vi "Migrate Measurements.vi"() -> ()   [LabVIEW 2021]
uses:
  _Measurement Migrator/Migrator/Queue Driver/controls/Queue Operations.ctl
  _Measurement Migrator/Migrator/Migration Logic/controls/Multiple Migration/Multiple Migration Data Holder.ctl
  <vilib>/Utility/sysdir.llb/System Directory Type.ctl
  <vilib>/Utility/miscctls.llb/LVRowAndColumnUnsignedTypeDef.ctl
  <vilib>/Utility/miscctls.llb/LVRowAndColumnTypeDef.ctl
  _Measurement Migrator/Migrator/Migrator Reusables/controls/Dictionary States.ctl
  <vilib>/Utility/cursorutil.llb/Set Cursor (Icon Pict).vi
  _Measurement Migrator/Migrator/Queue Driver/Queue Driver.lvlib
  _Measurement Migrator/Migrator/Migration Logic/Migrator.lvlib
  _Measurement Migrator/Migrator/Path Functions/Path Functions.lvlib
  _Measurement Migrator/Migrator/Multiple Migrator/Multiple Migrator.lvlib
  _Measurement Migrator/Migrator/Migrator Reusables/Migrator Reusables.lvlib
panel:
  out "error out":errorcluster
  in  "Tab Control":T1(tab)
  in  "Info":string
  in  "Select Measurement":path
  out "Warning":bool=TRUE caption="Warning:\nMeasurement should be an existing VI or folder path"
  in  "Populate measurements":bool
  in  "Select Project":path=path "C:/Users/aishwarya.lakshmi/Documents/Measurement Plug-ins/Measurement"
  in  "Select all":bool
  in  "Back to Home":bool
  in  "List Plug-ins":bool
  in  "Select Measurements":string(tree)
  out "Selection warning":string="Atleast one measurement should be selected"
  out "Plug-in info":string="* Rename the Plug-in if required"
  out "Plug-in warning":string="Warning:\n1. Measurement plug-in name must be unique \n2. Plugin name cannot contain any of the following characters:\n         \\ / : * ? \" < > |"
  in  "Start Migration":bool
  in  "Back to Select":bool
  in  "List of Selected Measurements":i32(listbox)
  in  "Measurement Count":i32(slide)=6 caption="Migrating 1 of 1 measurement(s)" scale=0.0..100.0
  in  "Progress":i32(slide)=9 caption="Saving the project files..." scale=0.0..15.0
  in  "Review":bool
  in  "Migration Status":i32(listbox)
  in  "Back to Status":bool
  in  "Select Plug-in":string(combo) caption="Select Measurement plug-in to review"
  in  "Start Next":bool
  out "Launch Type Spec":string
  out "Launch Logic":string
  out "Launch UI":string
  # "* Project in which the measurement plug-in will be created"
  # "* Select a measurement vi or a folder containing measurements"
  # ".lvproj"
  # "Select the measurements to migrate"
  # "Review the Measurement:\n1. Review the Measurement UI. Click here to launch.\n2. Review the Measurement Logic VI. Click here to launch.\n3. Review the Type Specialization VI. Click here to launch."
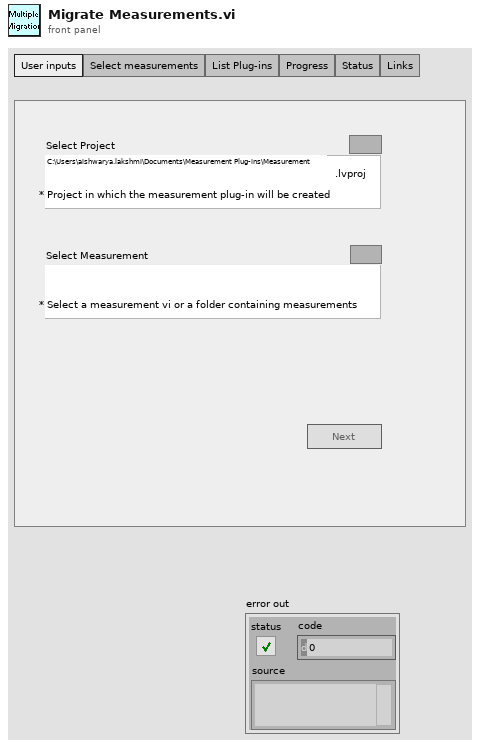
[diagram p1: front panel]
types:
  T1 = enum32{"User inputs", "Select measurements", "List Plug-ins", "Progress", "Status", "Links"}
  T2 = typedef "Queue Driver.lvlib/Queue Operations.ctl" = enum16{"Create Q", "Enqueue", "Enqueue N", "Dequeue", "Flush", "Release"}
  T3 = typedef "Migrator.lvlib/Multiple Migration Data Holder.ctl" = cluster{"Tree Reference":refnum<vi>, "LabVIEW Version":string, "Project path":path, "Create new project?":bool, "Measurement file/folder path":path, "Measurement folder selected?":bool, "Project warning":string, "Measurement warning":string, "Next clicked?":bool, "Measurement path changed?":bool, "Select all":bool, "Measurement folder Tags":string[], "Measurement file Tags":string[], "Selected cell Tag":string, "Measurement Plug-ins":string[][], "Measurement File Paths":path[], "Plugin Migration Value":i32, "Migration Count":i32, "Instrument containing subVIs":path[][], "Progress per measurement":i32, "Measurement Progress":i32, "Migration Status":string[][]}
  T4 = enum8{"Enabled", "Disabled", "Disabled and Grayed Out"}
  T5 = typedef "LVRowAndColumnUnsignedTypeDef.ctl" = cluster{"Row":u32, "Column":u32}
  T6 = typedef "LVRowAndColumnTypeDef.ctl" = cluster{"Row":i32, "Column":i32}
  T7 = typedef "Migrator Reusables.lvlib/Dictionary States.ctl" = enum16{"Set", "Get", "Delete", "Delete All"}
  T8 = typedef "System Directory Type.ctl" = i32
  T9 = typedef "LVPoint32TypeDef.ctl" = cluster{"Horizontal":i32, "Vertical":i32}
  T10 = typedef "Migrator.lvlib/Tree Items.ctl" = cluster{"Item name":string, "Indent":i32, "Tag":string}
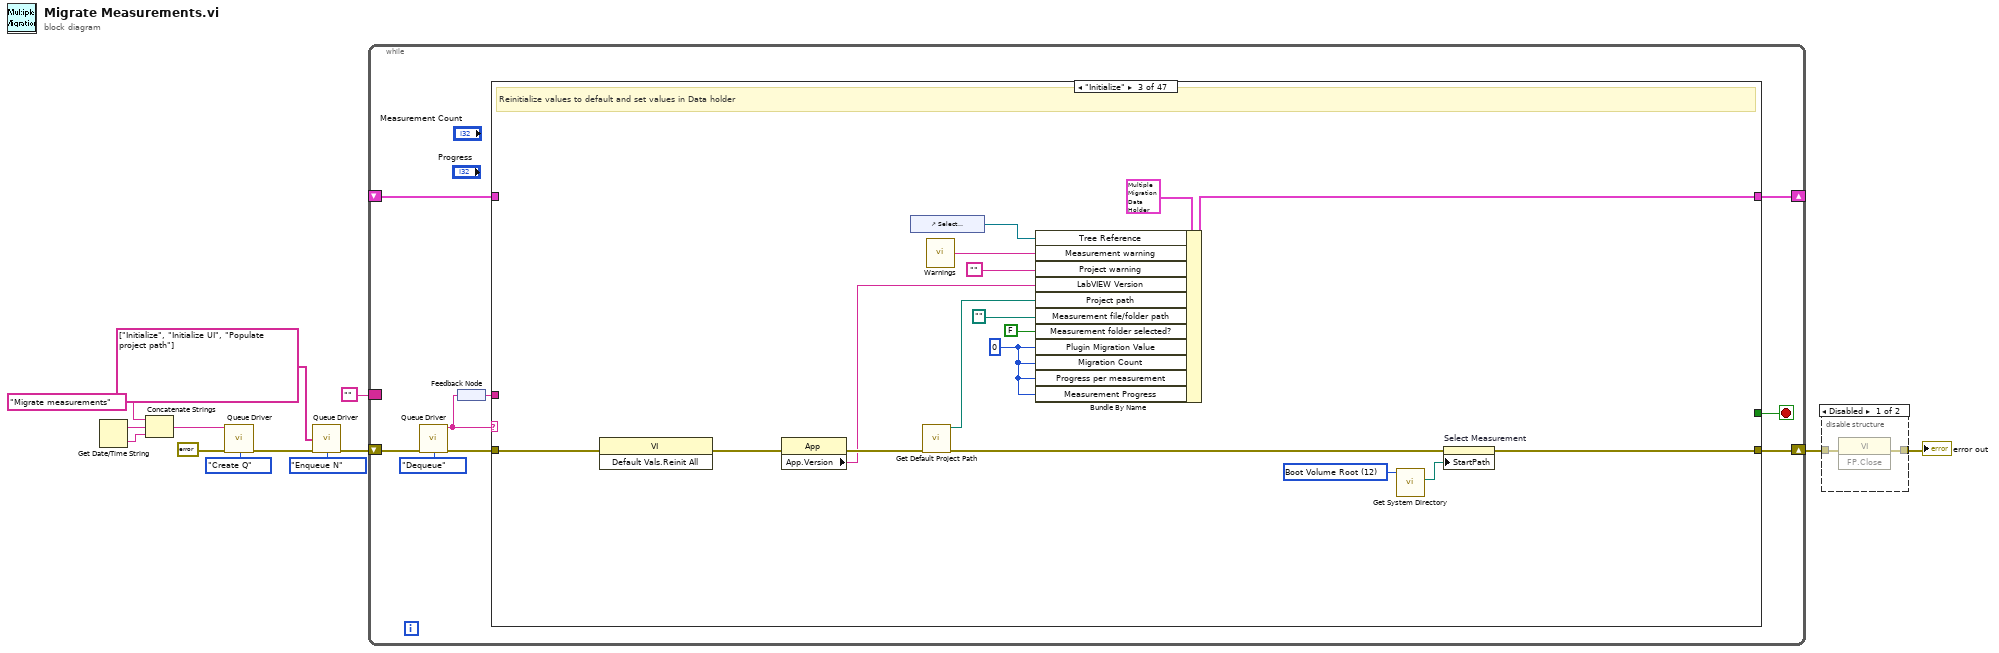
[diagram p0: block diagram]
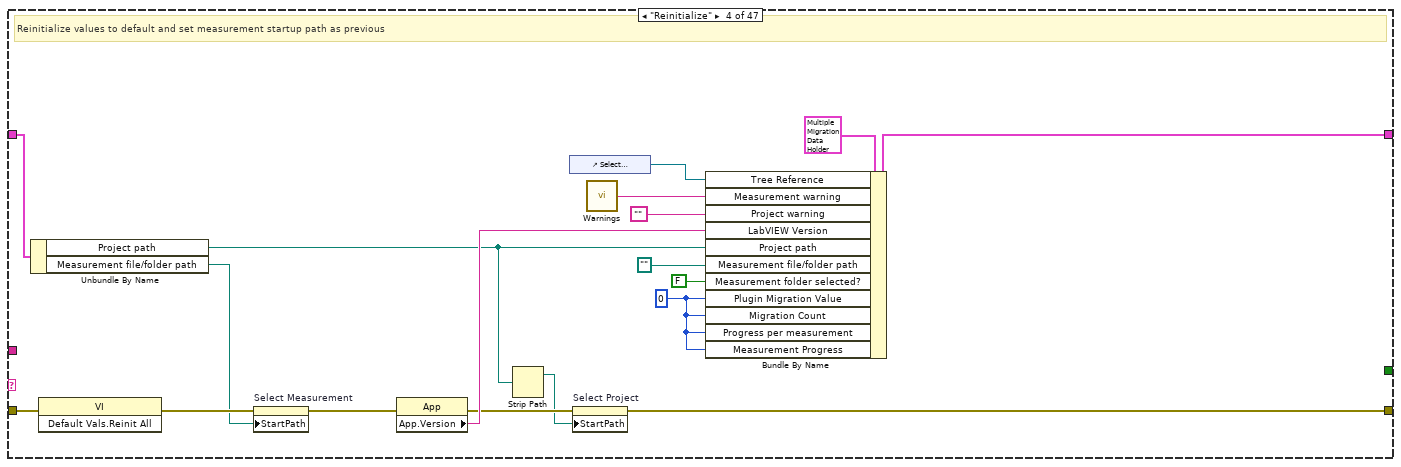
[diagram p5: hidden frame]
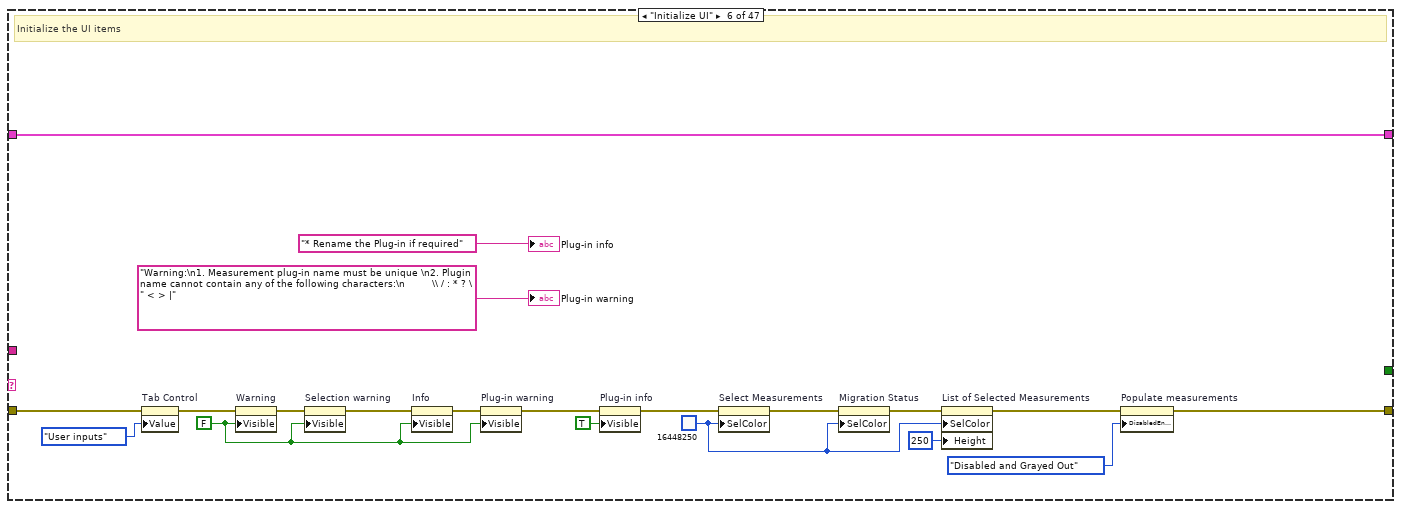
[diagram p7: hidden frame]
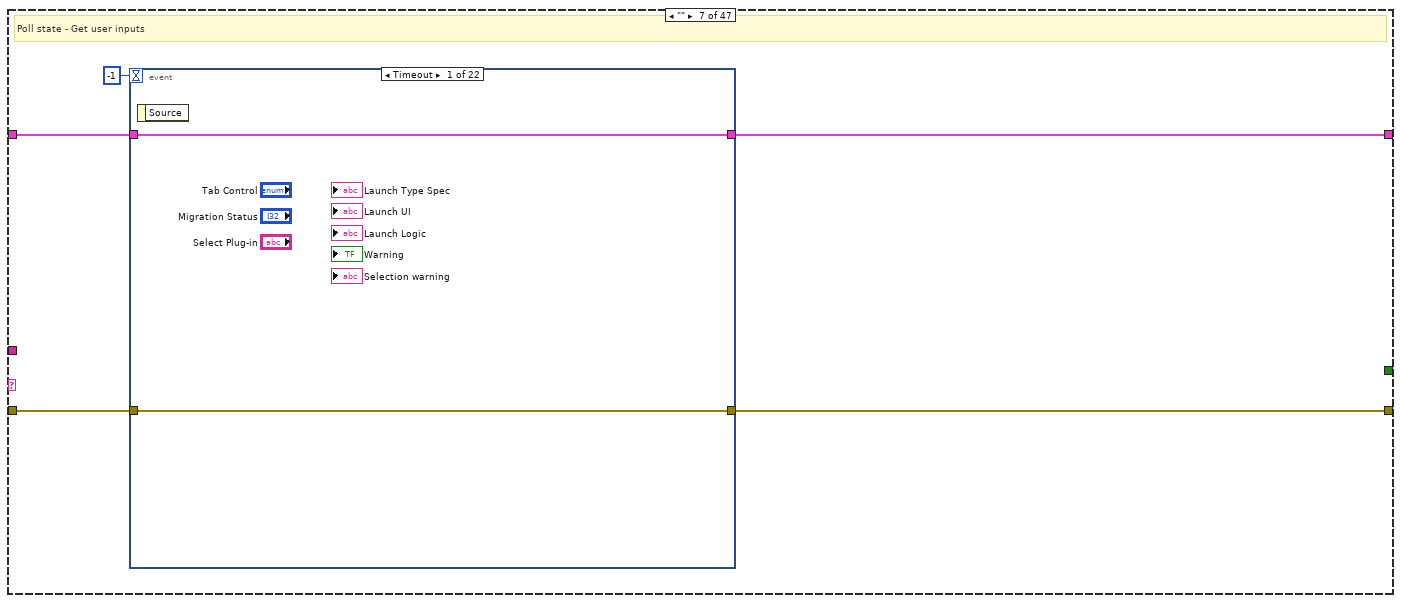
[diagram p8: hidden frame]
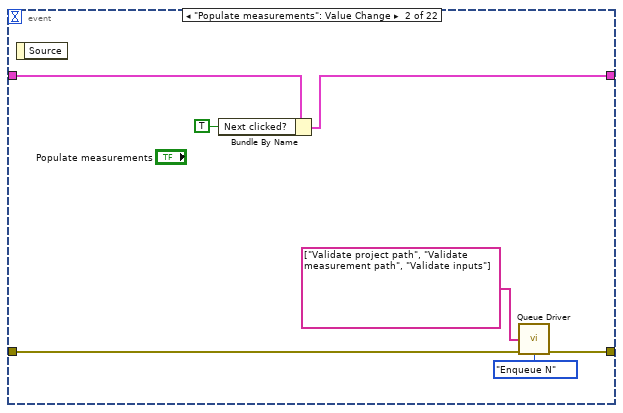
[diagram p9: hidden frame]
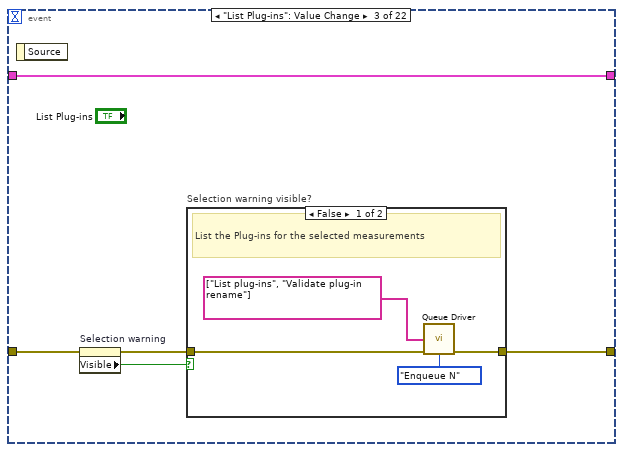
[diagram p10: hidden frame]
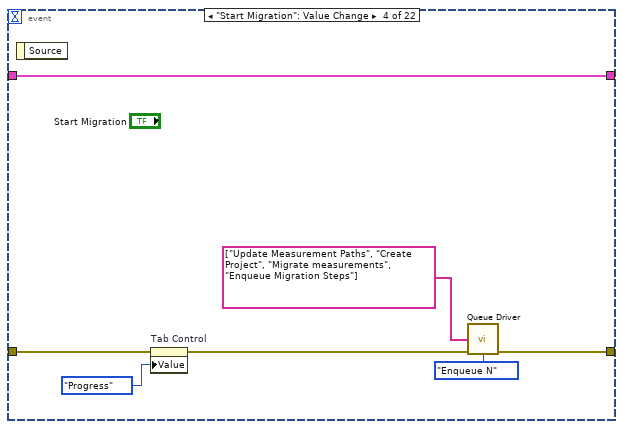
[diagram p12: hidden frame]
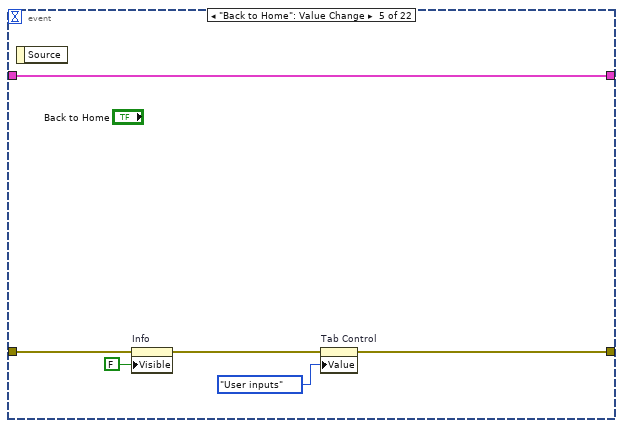
[diagram p13: hidden frame]
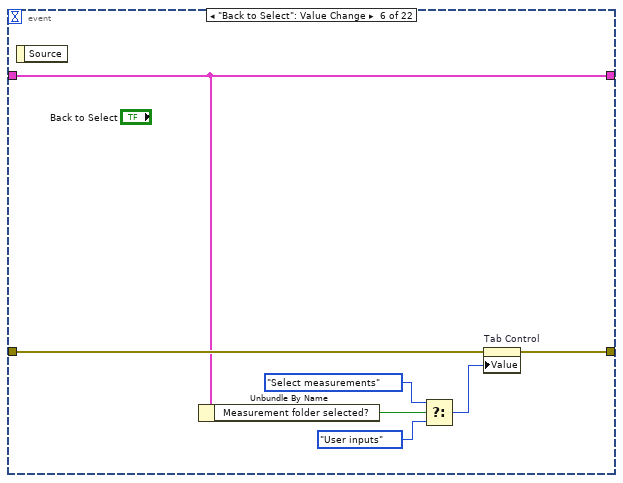
[diagram p14: hidden frame]
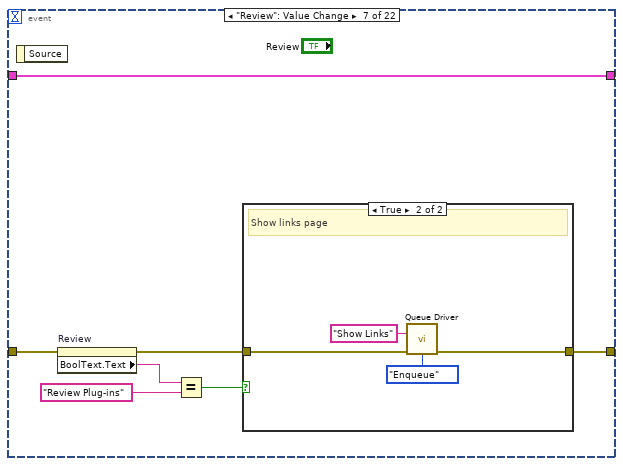
[diagram p15: hidden frame]
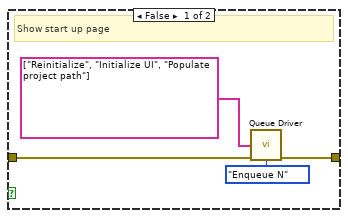
[diagram p16: hidden frame]
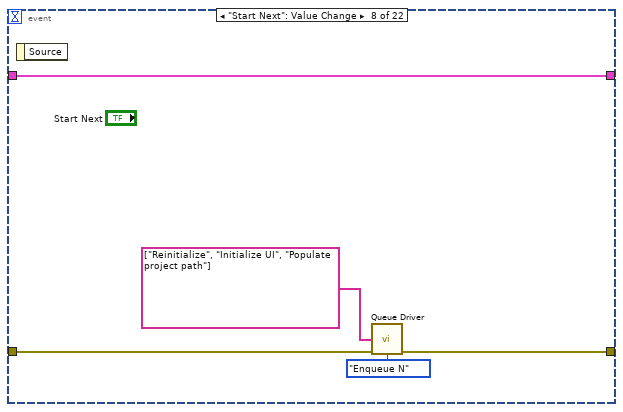
[diagram p17: hidden frame]
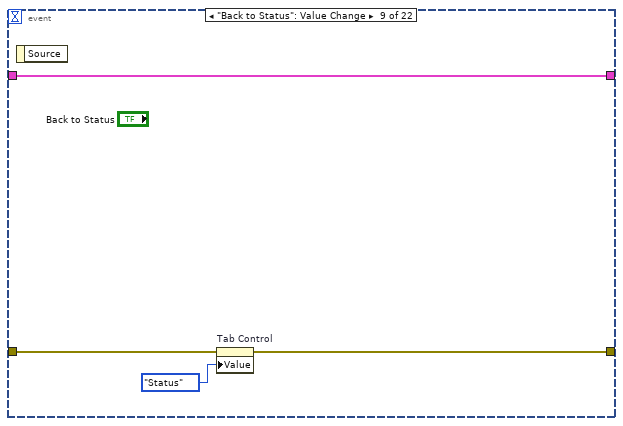
[diagram p18: hidden frame]
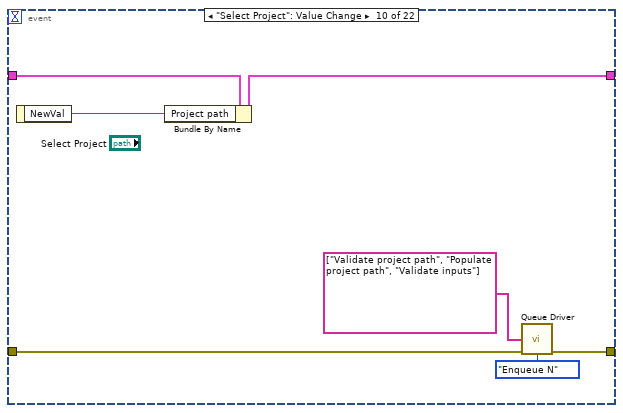
[diagram p19: hidden frame]
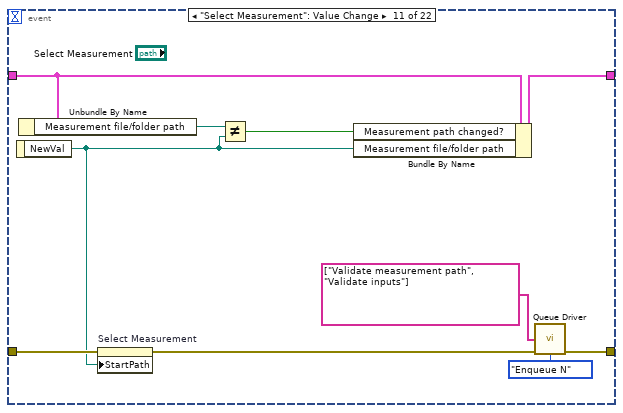
[diagram p20: hidden frame]
diagram:
  n1 = Get Date/Time String() -> (date string=w10:string, time string=w9:string)  [unwired: 3 in]
  n2 = Concatenate Strings("Migrate measurements" ("string"), w10, w9) -> (w4:string)
  n3 = call "Queue Driver.vi"("Name"=w4, "error in (no error)"=errorcluster {"status"=FALSE, "code"=0, "source"=""}, "Q Operations"=Queue_Operations."Create Q") -> ("error out"=w13:errorcluster)  [unwired: 11 in, 1 out]
  n4 = call "Queue Driver.vi"("States[]"=string[] ["Initialize", "Initialize UI", "Populate project path"], "error in (no error)"=w13, "Q Operations"=Queue_Operations."Enqueue N") -> ("error out"=w8:errorcluster)  [unwired: 11 in, 1 out]
  n5 = while {
    shift-right: [w21] -> w3
    shift-left: w8 -> [w22]
    shift-right: [w18] -> _
    shift-left: _ -> [w17]
    border: "" -> [_]
    stop <- w16 stop-if-true
    n6 = call "Queue Driver.vi"("error in (no error)"=w22, "Q Operations"=Queue_Operations."Dequeue") -> ("Dequeued State"=w15:string, "error out"=w20:errorcluster)  [unwired: 12 in]
    n7 = feedback #1() -> (w14:string)
    n8 = feedback-in #1(w15) -> ()
    n9 = case shown="\"Initialize\"" w15 {
      tunnel: w20 -> [w23 w26 w43 w61 w63 w83 w88 w260 w272 w283 w302 w326 w371 w388 w441 w466 w485 w543 w552 w558 w581 w591 w610 w627 w649 w656 w662 w668 w674 w680 w686 w692 w698 w704 w710 w716 w722 w728 w734 w756 w777 w789 w831 w840 w849 w870 w882]
      tunnel: [w23 w26 w32 w46 w63 w74 w87 w262 w272 w275 w301 w325 w371 w383 w429 w449 w472 w533 w552 w553 w578 w594 w609 w626 w648 w658 w664 w670 w676 w682 w688 w694 w700 w706 w712 w718 w724 w729 w738 w760 w777 w788 w828 w840 w846 w870 w872] -> w21
      tunnel: [w24 w25 w42 w60 w62 w79 w84 w261 w273 w278 w295 w313 w372 w389 w432 w464 w469 w538 w551 w573 w589 w603 w613 w646 w654 w660 w666 w672 w678 w684 w690 w696 w702 w708 w714 w720 w726 w732 w739 w761 w778 w793 w830 w841 w851 w871 w880] -> w18
      tunnel: w17 -> [w24 w25 _ w49 w62 w79 w85 w261 w273 w279 w297 w324 w372 w390 w433 w465 w470 w539 w551 w574 w589 w602 w613 w646 w654 w660 w666 w672 w678 w684 w690 w696 w702 w708 w714 w720 w726 w732 w740 w762 w778 w794 w830 w841 w851 w871 w880]
      tunnel: [_ _ _ _ _ _ _ _ _ _ _ _ _ _ _ _ _ _ _ _ _ _ _ _ _ _ _ _ _ _ _ _ _ _ _ _ _ _ _ _ _ _ _ _ _ _ TRUE] -> w16
      tunnel: w14 -> [_ _ _ _ _ _ _ _ _ _ _ _ _ _ _ _ _ _ _ _ _ _ _ _ _ _ _ _ _ _ _ _ _ _ _ _ _ _ _ _ _ _ _ _ w842 _ _]
      frame Default {
        # "Default case"
      }
      frame "/**********INITIALIZE**********/" {
      }
      frame "Initialize" {
        w27 = 0 ("Plugin Migration Value")
        w31 = T8 12 items=["User Home"=0, "User Desktop"=1, "User Documents"=2, "User Application Data"=3, "User Preferences"=4, "User Temporary"=5, "Public Documents"=6, "Public Application Data"=7, "Public Preferences"=8, "Public Cache"=13, "System Core Libraries"=9, "System Installed Libraries"=10, "Application Files"=11, "Boot Volume Root"=12] ("system directory type")
        # "Reinitialize values to default and set values in Data holder"
        n10 = invoke class="VI" method="Default Vals.Reinit All"(error in=w43) -> (error out=w40:errorcluster)  [unwired: 2 in, 2 out]
        n11 = property class="App"(error in=w40) -> (error out=w39:errorcluster, "App.Version"=w38:string)  [unwired: 1 in, 1 out]
        n12 = control-ref of="Select Measurements"() -> (w35:refnum<vi>)
        n13 = call "Get Default Project Path.vi"("error in"=w39) -> ("Project Path"=w41:path, "error out"=w33:errorcluster)  [unwired: 13 in]
        n14 = call "Warnings.vi"() -> ("Invalid measurement path"=w34:string)  [unwired: 8 in, 7 out]
        n15 = Bundle By Name(cluster=T3 {"Tree Reference"=refnum, "LabVIEW Version"="", "Project path"=path "", "Create new project?"=FALSE, "Measurement file/folder path"=path "", "Measurement folder selected?"=FALSE, "Project warning"="", "Measurement warning"="", "Next clicked?"=FALSE, "Measurement path changed?"=FALSE, "Select all"=FALSE, "Measurement folder Tags"=[], "Measurement file Tags"=[], "Selected cell Tag"="", "Measurement Plug-ins"=[], "Measurement File Paths"=[], "Plugin Migration Value"=0, "Migration Count"=0, "Instrument containing subVIs"=[], "Progress per measurement"=0, "Measurement Progress"=0, "Migration Status"=[]}, "Tree Reference"=w35, "Measurement warning"=w34, "Project warning"="", "LabVIEW Version"=w38, "Project path"=w41, "Measurement file/folder path"=path "", "Measurement folder selected?"=FALSE, "Plugin Migration Value"=w27, "Migration Count"=w27, "Progress per measurement"=w27, "Measurement Progress"=w27) -> (w42:T3)
        n16 = call <vilib>:"Get System Directory.vi"("system directory type"=w31) -> ("system directory"=w30:path)  [unwired: 10 in]
        n17 = property on="Select Measurement" class="Path"(error in=w33, "StartPath"=w30) -> (error out=w32:errorcluster)  [unwired: 1 in, 1 out]
      }
      frame "Reinitialize" {
        w52 = 0 ("Plugin Migration Value")
        # "Reinitialize values to default and set measurement startup path as previous"
        n18 = Unbundle By Name(w49) -> ("Project path"=w45:path, "Measurement file/folder path"=w48:path)
        n19 = invoke class="VI" method="Default Vals.Reinit All"(error in=w61) -> (error out=w51:errorcluster)  [unwired: 2 in, 2 out]
        n20 = property on="Select Measurement" class="Path"(error in=w51, "StartPath"=w48) -> (error out=w50:errorcluster)  [unwired: 1 in, 1 out]
        n21 = property class="App"(error in=w50) -> (error out=w47:errorcluster, "App.Version"=w59:string)  [unwired: 1 in, 1 out]
        n22 = Strip Path(path=w45) -> (stripped path=w44:path)  [unwired: 1 out]
        n23 = control-ref of="Select Measurements"() -> (w56:refnum<vi>)
        n24 = property on="Select Project" class="Path"(error in=w47, "StartPath"=w44) -> (error out=w46:errorcluster)  [unwired: 1 in, 1 out]
        n25 = call "Warnings.vi"() -> ("Invalid measurement path"=w55:string)  [unwired: 8 in, 7 out]
        n26 = Bundle By Name(cluster=T3 {"Tree Reference"=refnum, "LabVIEW Version"="", "Project path"=path "", "Create new project?"=FALSE, "Measurement file/folder path"=path "", "Measurement folder selected?"=FALSE, "Project warning"="", "Measurement warning"="", "Next clicked?"=FALSE, "Measurement path changed?"=FALSE, "Select all"=FALSE, "Measurement folder Tags"=[], "Measurement file Tags"=[], "Selected cell Tag"="", "Measurement Plug-ins"=[], "Measurement File Paths"=[], "Plugin Migration Value"=0, "Migration Count"=0, "Instrument containing subVIs"=[], "Progress per measurement"=0, "Measurement Progress"=0, "Migration Status"=[]}, "Tree Reference"=w56, "Measurement warning"=w55, "Project warning"="", "LabVIEW Version"=w59, "Project path"=w45, "Measurement file/folder path"=path "", "Measurement folder selected?"=FALSE, "Plugin Migration Value"=w52, "Migration Count"=w52, "Progress per measurement"=w52, "Measurement Progress"=w52) -> (w60:T3)
      }
      frame "/**********FP RELATED**********/" {
      }
      frame "Initialize UI" {
        w68 = FALSE ("Visible")
        w76 = u32 16448250 ("Selection Color")
        # "Initialize the UI items"
        n27 = property on="Tab Control" class="TabCtl (strict)"(error in=w83, "Value"=T1."User inputs" ("Tab Control")) -> (error out=w78:errorcluster)  [unwired: 1 in, 1 out]
        n28 = property on="Warning" class="Bool"(error in=w78, "Visible"=w68) -> (error out=w77:errorcluster)  [unwired: 1 in, 1 out]
        n29 = property on="Selection warning" class="Str"(error in=w77, "Visible"=w68) -> (error out=w72:errorcluster)  [unwired: 1 in, 1 out]
        n30 = property on="Info" class="Str"(error in=w72, "Visible"=w68) -> (error out=w71:errorcluster)  [unwired: 1 in, 1 out]
        n31 = property on="Plug-in warning" class="Str"(error in=w71, "Visible"=w68) -> (error out=w67:errorcluster)  [unwired: 1 in, 1 out]
        n32 = property on="Plug-in info" class="Str"(error in=w67, "Visible"=TRUE) -> (error out=w66:errorcluster)  [unwired: 1 in, 1 out]
        n33 = property on="Select Measurements" class="Tree (strict)"(error in=w66, "SelColor"=w76) -> (error out=w81:errorcluster)  [unwired: 1 in, 1 out]
        n34 = property on="Migration Status" class="MCListbox (strict)"(error in=w81, "SelColor"=w76) -> (error out=w80:errorcluster)  [unwired: 1 in, 1 out]
        n35 = property on="List of Selected Measurements" class="MCListbox (strict)"(error in=w80, "SelColor"=w76, "Height"=u32 250 ("Size:Height")) -> (error out=w75:errorcluster)  [unwired: 1 in, 1 out]
        n36 = property on="Populate measurements" class="Bool"(error in=w75, "DisabledEnum"=T4."Disabled and Grayed Out" ("Disabled")) -> (error out=w74:errorcluster)  [unwired: 1 in, 1 out]
        "Plug-in warning" <- "Warning:\n1. Measurement plug-in name must be unique \n2. Plugin name cannot contain any of the following characters:\n         \\ / : * ? \" < > |" ("f")
        "Plug-in info" <- "* Rename the Plug-in if required" ("Plug-in warning")
      }
      frame "" {
        # "Poll state - Get user inputs"
        n37 = event shown="[0] Timeout" {
          selector: _ -> [_ _ _ _ _ _ _ _ _ _ _ _ _ _ _ _ _ _ _ _ _ _]
          dyn-events: _ -> [_ _ _ _ _ _ _ _ _ _ _ _ _ _ _ _ _ _ _ _ _ _]
          timeout: -1 -> [_ _ _ _ _ _ _ _ _ _ _ _ _ _ _ _ _ _ _ _ _ _]
          tunnel: w88 -> [w90 w97 w100 w114 w117 w127 w131 w144 w151 w158 w164 w172 w183 w192 w200 w207 w210 w214 w220 w230 w242 w254]
          tunnel: [w90 w96 w101 w110 w120 w126 w133 w145 w150 w157 w167 w171 w178 w191 w198 w208 w211 w215 w222 w233 w244 w253] -> w87
          tunnel: w85 -> [w89 w93 w102 w111 w118 w125 w134 w147 w148 w155 w162 w175 w182 w193 w201 w209 w213 w217 w223 w234 w245 w255]
          tunnel: [w89 w92 w102 w111 w118 w125 w134 w147 w148 w154 w168 w174 w181 w193 w201 w209 w213 w217 w223 w234 w245 w255] -> w84
          event Timeout {
            # "Timeout"
            n38 = event-data() -> ()  [unwired: 1 in, 1 out]
          }
          event "Populate measurements": Value Change {
            n39 = event-data() -> ()  [unwired: 1 in, 1 out]
            n40 = Bundle By Name(cluster=w93, "Next clicked?"=TRUE) -> (w92:T3)
            n41 = call "Queue Driver.vi"("States[]"=string[] ["Validate project path", "Validate measurement path", "Validate inputs"], "error in (no error)"=w97, "Q Operations"=Queue_Operations."Enqueue N") -> ("error out"=w96:errorcluster)  [unwired: 11 in, 1 out]
          }
          event "List Plug-ins": Value Change {
            n42 = event-data() -> ()  [unwired: 1 in, 1 out]
            n43 = property on="Selection warning" class="Str"(error in=w100) -> (error out=w99:errorcluster, "Visible"=w98:bool)  [unwired: 1 in, 1 out]
            n44 = case "Selection warning visible?" shown="False" w98 {
              tunnel: w99 -> [w106 w107]
              tunnel: [w105 w107] -> w101
              frame False {
                # "List the Plug-ins for the selected measurements"
                n45 = call "Queue Driver.vi"("States[]"=string[] ["List plug-ins", "Validate plug-in rename"], "error in (no error)"=w106, "Q Operations"=Queue_Operations."Enqueue N") -> ("error out"=w105:errorcluster)  [unwired: 11 in, 1 out]
              }
              frame True {
                # "Pass"
              }
            }
          }
          event "Start Migration": Value Change {
            n46 = event-data() -> ()  [unwired: 1 in, 1 out]
            n47 = property on="Tab Control" class="TabCtl (strict)"(error in=w114, "Value"=T1."Progress" ("Tab Control")) -> (error out=w113:errorcluster)  [unwired: 1 in, 1 out]
            n48 = call "Queue Driver.vi"("States[]"=string[] ["Update Measurement Paths", "Create Project", "Migrate measurements", "Enqueue Migration Steps"], "error in (no error)"=w113, "Q Operations"=Queue_Operations."Enqueue N") -> ("error out"=w110:errorcluster)  [unwired: 11 in, 1 out]
          }
          event "Back to Home": Value Change {
            n49 = event-data() -> ()  [unwired: 1 in, 1 out]
            n50 = property on="Info" class="Str"(error in=w117, "Visible"=FALSE) -> (error out=w116:errorcluster)  [unwired: 1 in, 1 out]
            n51 = property on="Tab Control" class="TabCtl (strict)"(error in=w116, "Value"=T1."User inputs" ("Tab Control")) -> (error out=w120:errorcluster)  [unwired: 1 in, 1 out]
          }
          event "Back to Select": Value Change {
            n52 = event-data() -> ()  [unwired: 1 in, 1 out]
            n53 = Unbundle By Name(w125) -> ("Measurement folder selected?"=w124:bool)
            n54 = Select(t=T1."Select measurements" ("Tab Control"), s=w124, f=T1."User inputs" ("Tab Control")) -> (s? t:f=w121:T1)
            n55 = property on="Tab Control" class="TabCtl (strict)"(error in=w127, "Value"=w121) -> (error out=w126:errorcluster)  [unwired: 1 in, 1 out]
          }
          event "Review": Value Change {
            n56 = event-data() -> ()  [unwired: 1 in, 1 out]
            n57 = property on="Review" class="Bool"(error in=w131) -> (error out=w132:errorcluster, "BoolText.Text"=w130:string)  [unwired: 1 in, 1 out]
            n58 = Equal?(x=w130, y="Review Plug-ins") -> (x = y?=w128:bool)
            n59 = case shown="True" w128 {
              tunnel: [w136 w142] -> w133
              tunnel: w132 -> [w135 w139]
              frame False {
                # "Show start up page"
                n60 = call "Queue Driver.vi"("States[]"=string[] ["Reinitialize", "Initialize UI", "Populate project path"], "error in (no error)"=w135, "Q Operations"=Queue_Operations."Enqueue N") -> ("error out"=w136:errorcluster)  [unwired: 11 in, 1 out]
              }
              frame True {
                # "Show links page"
                n61 = call "Queue Driver.vi"("State"="Show Links", "error in (no error)"=w139, "Q Operations"=Queue_Operations."Enqueue") -> ("error out"=w142:errorcluster)  [unwired: 11 in, 1 out]
              }
            }
          }
          event "Start Next": Value Change {
            n62 = event-data() -> ()  [unwired: 1 in, 1 out]
            n63 = call "Queue Driver.vi"("States[]"=string[] ["Reinitialize", "Initialize UI", "Populate project path"], "error in (no error)"=w144, "Q Operations"=Queue_Operations."Enqueue N") -> ("error out"=w145:errorcluster)  [unwired: 11 in, 1 out]
          }
          event "Back to Status": Value Change {
            n64 = event-data() -> ()  [unwired: 1 in, 1 out]
            n65 = property on="Tab Control" class="TabCtl (strict)"(error in=w151, "Value"=T1."Status" ("Tab Control")) -> (error out=w150:errorcluster)  [unwired: 1 in, 1 out]
          }
          event "Select Project": Value Change {
            n66 = event-data() -> ("NewVal"=w153:path)  [unwired: 1 in]
            n67 = Bundle By Name(cluster=w155, "Project path"=w153) -> (w154:T3)
            n68 = call "Queue Driver.vi"("States[]"=string[] ["Validate project path", "Populate project path", "Validate inputs"], "error in (no error)"=w158, "Q Operations"=Queue_Operations."Enqueue N") -> ("error out"=w157:errorcluster)  [unwired: 11 in, 1 out]
          }
          event "Select Measurement": Value Change {
            n69 = event-data() -> ("NewVal"=w159:path)  [unwired: 1 in]
            n70 = Unbundle By Name(w162) -> ("Measurement file/folder path"=w160:path)
            n71 = property on="Select Measurement" class="Path"(error in=w164, "StartPath"=w159) -> (error out=w163:errorcluster)  [unwired: 1 in, 1 out]
            n72 = Not Equal?(x=w160, y=w159) -> (x != y?=w161:bool)
            n73 = Bundle By Name(cluster=w162, "Measurement path changed?"=w161, "Measurement file/folder path"=w159) -> (w168:T3)
            n74 = call "Queue Driver.vi"("States[]"=string[] ["Validate measurement path", "Validate inputs"], "error in (no error)"=w163, "Q Operations"=Queue_Operations."Enqueue N") -> ("error out"=w167:errorcluster)  [unwired: 11 in, 1 out]
          }
          event "Select all": Value Change {
            n75 = event-data() -> ("NewVal"=w173:bool)  [unwired: 1 in]
            n76 = Bundle By Name(cluster=w175, "Select all"=w173) -> (w174:T3)
            n77 = call "Queue Driver.vi"("State"="Select/Deselect all", "error in (no error)"=w172, "Q Operations"=Queue_Operations."Enqueue") -> ("error out"=w171:errorcluster)  [unwired: 11 in, 1 out]
          }
          event "Select Measurements": Mouse Down {
            n78 = event-data() -> ("Coords"=w176:T9)  [unwired: 1 in]
            n79 = invoke on="Select Measurements" class="Tree (strict)" method="Point To Row Column"(error in=w183, "Point"=w176) -> (error out=w179:errorcluster, "Tag"=w180:string, "InGlyph"=w177:bool)  [unwired: 6 in, 5 out]
            n80 = case "In Symbol?" shown="True" w177 {
              tunnel: w179 -> [w184 w188]
              tunnel: [w184 w187] -> w178
              frame False {
                # "Pass"
              }
              frame True {
                # "Update the selection of measurements"
                n81 = call "Queue Driver.vi"("State"="Measurement selection" ("State 2"), "error in (no error)"=w188, "Q Operations"=Queue_Operations."Enqueue") -> ("error out"=w187:errorcluster)  [unwired: 11 in, 1 out]
              }
            }
            n82 = Bundle By Name(cluster=w182, "Selected cell Tag"=w180) -> (w181:T3)
          }
          event "List of Selected Measurements": Edit Cell {
            n83 = event-data() -> ()  [unwired: 1 in, 1 out]
            n84 = call "Queue Driver.vi"("State"="Validate plug-in rename", "error in (no error)"=w192, "Q Operations"=Queue_Operations."Enqueue") -> ("error out"=w191:errorcluster)  [unwired: 11 in, 1 out]
          }
          event "List of Selected Measurements": Mouse Down {
            n85 = event-data() -> ("Coords"=w197:T9)  [unwired: 1 in, 7 out]
            n86 = invoke on="List of Selected Measurements" class="MCListbox (strict)" method="Point To Row Column"(error in=w200, "Point"=w197) -> (error out=w199:errorcluster, "CellPosition"=w194:T6)  [unwired: 5 in, 5 out]
            n87 = Unbundle By Name(w194) -> ("Column"=w196:i32)
            n88 = Not Equal To 0?(x=w196) -> (x != 0?=w195:bool)
            n89 = case shown="False" w195 {
              tunnel: w199 -> [w202 w205]
              tunnel: [w202 w204] -> w198
              tunnel: w194 -> [_ w203]
              frame False {
              }
              frame True {
                n90 = property on="List of Selected Measurements" class="MCListbox (strict)"(error in=w205, "EditPos"=w203) -> (error out=w204:errorcluster)  [unwired: 1 in, 1 out]
              }
            }
          }
          event "Select Plug-in": Value Change {
            n91 = event-data() -> ("NewVal"=w206:string)  [unwired: 1 in]
            n92 = call "Set Measurement Name.vi"("Name"=w206, "error in (no error)"=w207) -> ("error out"=w208:errorcluster)  [unwired: 13 in]
          }
          event "Launch UI", "Launch Logic", "Launch Type Spec": Mouse Enter {
            n93 = event-data() -> ()  [unwired: 1 in, 1 out]
            n94 = call-poly <vilib>:"Set Cursor.vi"("error in (no error)"=w210, "icon"=u16 6) -> ("error out"=w211:errorcluster)  [unwired: 8 in, 1 out]
          }
          event "Launch UI", "Launch Logic", "Launch Type Spec": Mouse Leave {
            n95 = event-data() -> ()  [unwired: 1 in, 1 out]
            n96 = call-poly <vilib>:"Set Cursor.vi"("error in (no error)"=w214, "icon"=u16 0) -> ("error out"=w215:errorcluster)  [unwired: 8 in, 1 out]
          }
          event "Launch UI": Mouse Down {
            n97 = event-data() -> ()  [unwired: 1 in, 1 out]
            n98 = property on="Select Plug-in" class="CmbBox"(error in=w220) -> (error out=w221:errorcluster, "Value"=w219:string)  [unwired: 1 in, 1 out]
            n99 = Empty String/Path?(string/path=w219) -> (empty?=w218:bool)
            n100 = case shown="False" w218 {
              tunnel: [w226 w228] -> w222
              tunnel: w221 -> [w224 w228]
              frame False {
                n101 = call "Measurement Plugin Path.vi"("error in (no error)"=w224) -> ("Measurement UI"=w225:path, "error out"=w227:errorcluster)  [unwired: 2 in, 11 out]
                n102 = call "Open VI.vi"("Logic VI Path"=w225, "error in (no error)"=w227) -> ("error out"=w226:errorcluster)  [unwired: 13 in]
              }
              frame True {
              }
            }
          }
          event "Launch Logic": Mouse Down {
            n103 = event-data() -> ()  [unwired: 1 in, 1 out]
            n104 = property on="Select Plug-in" class="CmbBox"(error in=w230) -> (error out=w231:errorcluster, "Value"=w232:string)  [unwired: 1 in, 1 out]
            n105 = Empty String/Path?(string/path=w232) -> (empty?=w229:bool)
            n106 = case shown="False" w229 {
              tunnel: [w237 w239] -> w233
              tunnel: w231 -> [w236 w239]
              frame False {
                n107 = call "Measurement Plugin Path.vi"("error in (no error)"=w236) -> ("Logic VI Path"=w235:path, "error out"=w238:errorcluster)  [unwired: 2 in, 11 out]
                n108 = call "Open VI.vi"("Logic VI Path"=w235, "error in (no error)"=w238) -> ("error out"=w237:errorcluster)  [unwired: 13 in]
              }
              frame True {
              }
            }
          }
          event "Launch Type Spec": Mouse Down {
            n109 = event-data() -> ()  [unwired: 1 in, 1 out]
            n110 = property on="Select Plug-in" class="CmbBox"(error in=w242) -> (error out=w241:errorcluster, "Value"=w243:string)  [unwired: 1 in, 1 out]
            n111 = Empty String/Path?(string/path=w243) -> (empty?=w240:bool)
            n112 = case shown="False" w240 {
              tunnel: [w248 w250] -> w244
              tunnel: w241 -> [w247 w250]
              frame False {
                n113 = call "Measurement Plugin Path.vi"("error in (no error)"=w247) -> ("Type Specialization"=w246:path, "error out"=w249:errorcluster)  [unwired: 2 in, 11 out]
                n114 = call "Open VI.vi"("Logic VI Path"=w246, "error in (no error)"=w249) -> ("error out"=w248:errorcluster)  [unwired: 13 in]
              }
              frame True {
              }
            }
          }
          event Panel Close? {
            n115 = event-data() -> ()  [unwired: 1 in, 1 out]
            n116 = call "Queue Driver.vi"("State"="Exit", "error in (no error)"=w254, "Q Operations"=Queue_Operations."Enqueue") -> ("error out"=w253:errorcluster)  [unwired: 11 in, 1 out]
            n117 = event-data("Discard?"=TRUE) -> ()  [unwired: 1 in, 1 out]
          }
        }
      }
      frame "Populate project path" {
        # "Populate the validated project path in the control"
        n118 = Unbundle By Name(w261) -> ("Project warning"=w258:string, "Project path"=w259:path)
        n119 = Empty String/Path?(string/path=w258) -> (empty?=w257:bool)
        n120 = case "Valid project?" shown="True" w257 {
          tunnel: [w263 w271] -> w262
          tunnel: w260 -> [w263 w270]
          tunnel: w259 -> [_ w265]
          frame False {
            # "Pass"
          }
          frame True {
            # "Populate the path in the control"
            n121 = call <vilib>:"Get File Extension.vi"("error in (no error)"=w270, "file"=w265) -> ("error out"=w269:errorcluster, "filename without extension"=w268:string)  [unwired: 5 in, 3 out]
            n122 = Concatenate Strings("..\\" ("string"), w268) -> (w266:string)
            n123 = Build Path(base path=w265, name or relative path=w266) -> (appended path=w264:path)
            n124 = property on="Select Project" class="Path"(error in=w269, "Value"=w264) -> (error out=w271:errorcluster)  [unwired: 1 in, 1 out]
          }
        }
      }
      frame "/**********INPUT VALIDATION**********/" {
      }
      frame "Validate project path" {
        # "Validate the project path and set warning if required"
        n125 = Unbundle By Name(w279) -> ("Project path"=w280:path, "LabVIEW Version"=w281:string)
        n126 = call <vilib>:"Is Path and Not Empty.vi"("path"=w280) -> ("Is Path and Not Empty?"=w282:bool)  [unwired: 4 in]
        n127 = case "Is Path and not empty?" shown="True" w282 {
          tunnel: w283 -> [w286 w293]
          tunnel: [w286 w292] -> w275
          tunnel: [w284 w291] -> w274
          tunnel: w281 -> [_ w290]
          tunnel: w280 -> [w285 w289]
          tunnel: [_ w288] -> w277
          tunnel: [w285 w287] -> w276
          frame False {
            # "Set warning"
            n128 = call "Warnings.vi"() -> ("Invalid project path"=w284:string)  [unwired: 8 in, 7 out]
          }
          frame True {
            # "Validate the path"
            n129 = call "Validate Project Path.vi"("Project path in"=w289, "LabVIEW Version"=w290, "error in (no error)"=w293) -> ("Validated project path"=w287:path, "New project?"=w288:bool, "Warning"=w291:string, "error out"=w292:errorcluster)  [unwired: 9 in]
          }
        }
        n130 = Bundle By Name(cluster=w279, "Project path"=w276, "Create new project?"=w277, "Project warning"=w274) -> (w278:T3)
      }
      frame "Validate measurement path" {
        # "Validate the measurement path and set warning if required"
        n131 = Unbundle By Name(w297) -> ("Measurement file/folder path"=w299:path, "LabVIEW Version"=w300:string)
        n132 = call <vilib>:"Is Path and Not Empty.vi"("path"=w299) -> ("Is Path and Not Empty?"=w298:bool)  [unwired: 4 in]
        n133 = case "Is Path and not empty?" shown="True" w298 {
          tunnel: w302 -> [w304 w310]
          tunnel: w299 -> [_ w309]
          tunnel: w300 -> [_ w308]
          tunnel: [w304 w307] -> w301
          tunnel: [w303 w306] -> w294
          tunnel: [_ w305] -> w296
          frame False {
            # "Set warning"
            n134 = call "Warnings.vi"() -> ("Invalid measurement path"=w303:string)  [unwired: 8 in, 7 out]
          }
          frame True {
            # "Validate the path"
            n135 = call "Validate Measurement Path.vi"("Measurement path"=w309, "LabVIEW version"=w308, "error in (no error)"=w310) -> ("Folder?"=w305:bool, "Warning"=w306:string, "error out"=w307:errorcluster)  [unwired: 10 in]
          }
        }
        n136 = Bundle By Name(cluster=w297, "Measurement folder selected?"=w296, "Measurement warning"=w294) -> (w295:T3)
      }
      frame "Validate inputs" {
        # "Validate the project path and measurement path inputs"
        n137 = Unbundle By Name(w324) -> ("Project warning"=w318:string, "Measurement warning"=w323:string, "Next clicked?"=w319:bool, "Project warning"=w317:string, "Measurement warning"=w316:string, "Measurement folder selected?"=w315:bool, "Measurement path changed?"=w314:bool)
        n138 = Empty String/Path?(string/path=w323) -> (empty?=w322:bool)
        n139 = Empty String/Path?(string/path=w318) -> (empty?=w321:bool)
        n140 = And(x=w321, y=w322) -> (x .and. y?=w320:bool)
        n141 = case "Valid inputs?" shown="True" w320 {
          tunnel: w326 -> [w340 w350]
          tunnel: [w335 w346] -> w325
          tunnel: w319 -> [_ w344]
          tunnel: w317 -> [w328 _]
          tunnel: w316 -> [w331 _]
          tunnel: w315 -> [_ w343]
          tunnel: w314 -> [w327 w342]
          tunnel: [w327 w341] -> w311
          frame False {
            # "Set the appropriate warning"
            n142 = call "Edit Warning.vi"("Warning in"=w328) -> ("Warning out"=w330:string)  [unwired: 6 in]
            n143 = call "Edit Warning.vi"("Warning in"=w331) -> ("Warning out"=w329:string)  [unwired: 6 in]
            n144 = Concatenate Strings("Warning:" ("string"), "\n", w330, w329) -> (w333:string)
            n145 = call "Get Warning Position.vi"("Warning"=w333) -> ("Warning position"=w332:i32)  [unwired: 6 in]
            n146 = property on="Warning" class="Bool"(error in=w340, "Visible"=TRUE, "Caption.Text"=w333, "Caption.Top"=w332) -> (error out=w336:errorcluster)  [unwired: 1 in, 1 out]
            n147 = property on="Populate measurements" class="Bool"(error in=w336, "DisabledEnum"=T4."Disabled and Grayed Out" ("Disabled")) -> (error out=w335:errorcluster)  [unwired: 1 in, 1 out]
          }
          frame True {
            # "Check if next is clicked and make the warning invisible"
            n148 = case "Next clicked?" shown="True" w344 {
              tunnel: w350 -> [w352 w357]
              tunnel: [w352 w356] -> w349
              tunnel: w343 -> [_ w355]
              tunnel: w342 -> [w351 w354]
              tunnel: [w351 FALSE] -> w341
              frame False {
                # "Pass"
              }
              frame True {
                # "Populate measurements if folder is selected and List the plug-ins if not"
                n149 = case "Measurement path changed?" shown="True" w354 {
                  tunnel: w357 -> [w363 w370]
                  tunnel: [w362 w369] -> w356
                  tunnel: w355 -> [w358 w364]
                  frame False {
                    # "Measurement folder?"
                    n150 = Select(t=T1."Select measurements" ("Tab Control"), s=w358, f=T1."List Plug-ins" ("Tab Control")) -> (s? t:f=w359:T1)
                    n151 = property on="Tab Control" class="TabCtl (strict)"(error in=w363, "Value"=w359) -> (error out=w362:errorcluster)  [unwired: 1 in, 1 out]
                  }
                  frame True {
                    # "Measurement folder?"
                    n152 = Select(t="Populate measurements" ("State 2"), s=w364, f="List plug-ins" ("State 2")) -> (s? t:f=w365:string)
                    n153 = call "Queue Driver.vi"("State"=w365, "error in (no error)"=w370, "Q Operations"=Queue_Operations."Enqueue") -> ("error out"=w369:errorcluster)  [unwired: 11 in, 1 out]
                  }
                }
              }
            }
            n154 = property on="Warning" class="Bool"(error in=w349, "Visible"=FALSE) -> (error out=w347:errorcluster)  [unwired: 1 in, 1 out]
            n155 = property on="Populate measurements" class="Bool"(error in=w347, "DisabledEnum"=T4."Enabled" ("Disabled")) -> (error out=w346:errorcluster)  [unwired: 1 in, 1 out]
          }
        }
        n156 = Bundle By Name(cluster=w324, "Next clicked?"=FALSE, "Measurement path changed?"=w311) -> (w313:T3)
      }
      frame "/**********FUNCTIONALITY**********/" {
      }
      frame "Populate measurements" {
        w377 = TRUE ("Visible")
        # "Populate the measurements in the Tree and set icon to the items"
        n157 = Unbundle By Name(w390) -> ("Tree Reference"=w384:refnum<vi>, "Measurement file/folder path"=w393:path, "LabVIEW Version"=w391:string)
        n158 = call "Set Cursor Icon.vi"("Cursor icon"=u16 2, "error in (no error)"=w388) -> ("error out"=w387:errorcluster)  [unwired: 13 in]
        n159 = property on="Info" class="Str"(error in=w387, "Visible"=w377, "Text.FontBold"=w377, "Text.Text"="Populating the measurements..." ("Info")) -> (error out=w386:errorcluster)  [unwired: 1 in, 1 out]
        n160 = call "Get Measurements.vi"("Input path"=w393, "LabVIEW version"=w391, "error in (no error)"=w386) -> ("Error?"=w378:string, "VI list"=w380:T10[], "Folder list"=w379:T10[], "error out"=w392:errorcluster)  [unwired: 9 in]
        n161 = Empty String/Path?(string/path=w378) -> (empty?=w381:bool)
        n162 = case "No error occured during get measurements?" shown="True" w381 {
          tunnel: w392 -> [w394 w426]
          tunnel: w390 -> [w401 w425]
          tunnel: [w400 w424] -> w389
          tunnel: w384 -> [w399 w423]
          tunnel: [w397 w422] -> w374
          tunnel: w380 -> [_ w413]
          tunnel: w379 -> [_ w412]
          tunnel: w378 -> [w398 _]
          frame False {
            # "Update the warning"
            n163 = Bundle By Name(cluster=w401, "Tree Reference"=w399, "Measurement warning"=w398) -> (w400:T3)
            n164 = call "Queue Driver.vi"("State"="Validate inputs", "error in (no error)"=w394, "Q Operations"=Queue_Operations."Enqueue") -> ("error out"=w397:errorcluster)  [unwired: 11 in, 1 out]
          }
          frame True {
            w411 = FALSE
            # "Populate the Tree with the measurements"
            n165 = call "Populate Tree.vi"("TreeControl in"=w423, "VI list"=w413, "Folder list"=w412, "error in (no error)"=w426) -> ("TreeControl out"=w420:refnum<vi>, "error out"=w421:errorcluster)  [unwired: 10 in]
            n166 = call "Set Tree Item Icon.vi"("TreeControl in"=w420, "error in (no error)"=w421) -> ("TreeControl out"=w416:refnum<vi>, "Measurement folder Tags"=w414:string[], "Measurement file Tags"=w415:string[], "error out"=w419:errorcluster)  [unwired: 10 in]
            n167 = Empty Array?(array=w415) -> (empty?=w404:bool)
            n168 = Select(t="No Measurement found in the folder" ("Warning"), s=w404, f="Atleast one measurement should be selected" ("Text.Text")) -> (s? t:f=w405:string)
            n169 = property on="Selection warning" class="Str"(error in=w419, "Visible"=TRUE, "Text.Text"=w405) -> (error out=w410:errorcluster)  [unwired: 1 in, 1 out]
            n170 = Select(t=T4."Disabled and Grayed Out" ("Disabled"), s=w404, f=T4."Enabled") -> (s? t:f=w403:T4)
            n171 = Bundle By Name(cluster=w425, "Tree Reference"=w416, "Measurement folder Tags"=w414, "Measurement file Tags"=w415, "Select all"=w411) -> (w424:T3)
            n172 = property on="Select all" class="Bool (strict)"(error in=w410, "Value"=w411, "DisabledEnum"=w403) -> (error out=w417:errorcluster)  [unwired: 1 in, 1 out]
            n173 = property on="Tab Control" class="TabCtl (strict)"(error in=w417, "Value"=T1."Select measurements" ("Tab Control")) -> (error out=w422:errorcluster)  [unwired: 1 in, 1 out]
          }
        }
        n174 = property on="Info" class="Str"(error in=w374, "Visible"=FALSE) -> (error out=w373:errorcluster)  [unwired: 1 in, 1 out]
        n175 = call "Set Cursor Icon.vi"("Cursor icon"=u16 0, "error in (no error)"=w373) -> ("error out"=w383:errorcluster)  [unwired: 13 in]
      }
      frame "Select/Deselect all" {
        # "Update the selection of items in the Tree based on the value of Select all"
        n176 = call "Set Cursor Icon.vi"("Cursor icon"=u16 2, "error in (no error)"=w441) -> ("error out"=w430:errorcluster)  [unwired: 13 in]
        n177 = Unbundle By Name(w433) -> ("Tree Reference"=w434:refnum<vi>, "Measurement folder Tags"=w436:string[], "Measurement file Tags"=w438:string[], "Select all"=w440:bool)
        n178 = Not(x=w440) -> (.not. x?=w442:bool)
        n179 = call "Tree Icons.vi"() -> ("Not Selected"=w444:i32, "Selected"=w445:i32)  [unwired: 6 in]
        n180 = property on="Selection warning" class="Str"(error in=w430, "Text.Text"="Atleast one measurement should be selected", "Visible"=w442) -> (error out=w439:errorcluster)  [unwired: 1 in, 1 out]
        n181 = Select(t=w445, s=w440, f=w444) -> (s? t:f=w437:i32)
        n182 = call "Update Tree Item Icon.vi"("TreeControl in"=w434, "Measurement folder Tags"=w436, "Measurement file Tags"=w438, "Icon"=w437, "error in (no error)"=w439) -> ("TreeControl out"=w431:refnum<vi>, "error out"=w435:errorcluster)  [unwired: 9 in]
        n183 = Bundle By Name(cluster=w433, "Tree Reference"=w431) -> (w432:T3)
        n184 = call "Set Cursor Icon.vi"("Cursor icon"=u16 0, "error in (no error)"=w435) -> ("error out"=w429:errorcluster)  [unwired: 13 in]
      }
      frame "Measurement selection" {
        # "Update the icons of the Tree items based on the selection"
        n185 = call "Set Cursor Icon.vi"("Cursor icon"=u16 2, "error in (no error)"=w466) -> ("error out"=w451:errorcluster)  [unwired: 13 in]
        n186 = Unbundle By Name(w465) -> ("Tree Reference"=w446:refnum<vi>, "Measurement folder Tags"=w456:string[], "Measurement file Tags"=w455:string[], "Selected cell Tag"=w457:string)
        n187 = call "Update Tree Item Selection.vi"("TreeControl in"=w446, "Measurement folder Tags"=w456, "Measurement file Tags"=w455, "Selected cell Tag"=w457, "error in (no error)"=w451) -> ("TreeControl out"=w452:refnum<vi>, "error out"=w462:errorcluster)  [unwired: 9 in]
        n188 = Insert Into Array(array=w456, new element=w455) -> (w458:string[])  [unwired: 1 in]
        n189 = call "Verify Select All.vi"("TreeControl in"=w452, "Measurement Tags"=w458, "error in (no error)"=w462) -> ("TreeControl out"=w454:refnum<vi>, "Select"=w447:bool, "Deselect"=w453:bool, "error out"=w461:errorcluster)  [unwired: 9 in]
        n190 = Bundle By Name(cluster=w465, "Tree Reference"=w454, "Select all"=w447) -> (w464:T3)
        n191 = property on="Select all" class="Bool (strict)"(error in=w461, "Value"=w447) -> (error out=w460:errorcluster)  [unwired: 1 in, 1 out]
        n192 = property on="Selection warning" class="Str"(error in=w460, "Text.Text"="Atleast one measurement should be selected", "Visible"=w453) -> (error out=w463:errorcluster)  [unwired: 1 in, 1 out]
        n193 = call "Set Cursor Icon.vi"("Cursor icon"=u16 0, "error in (no error)"=w463) -> ("error out"=w449:errorcluster)  [unwired: 13 in]
      }
      frame "List plug-ins" {
        # "List the Plug-in names of the selected measurements"
        n194 = Unbundle By Name(w470) -> ("Tree Reference"=w475:refnum<vi>, "Measurement file Tags"=w481:string[], "Measurement folder selected?"=w484:bool, "Measurement file/folder path"=w483:path)
        n195 = call "Set Cursor Icon.vi"("Cursor icon"=u16 2, "error in (no error)"=w485) -> ("error out"=w474:errorcluster)  [unwired: 13 in]
        n196 = case "Measurement Folder?" shown="True" w484 {
          tunnel: w474 -> [w500 w506]
          tunnel: w483 -> [w499 _]
          tunnel: [w498 w503] -> w482
          tunnel: [w496 w502] -> w468
          tunnel: w481 -> [_ w505]
          tunnel: w475 -> [w495 w504]
          tunnel: [w495 w501] -> w467
          frame False {
            # "Get the plug-in name of the selected measurement file"
            n197 = call <vilib>:"Get File Extension.vi"("error in (no error)"=w500, "file"=w499) -> ("error out"=w498:errorcluster, "filename without extension"=w494:string)  [unwired: 5 in, 3 out]
            n198 = Build Array(w494, w494) -> (w497:string[])
            n199 = Build Array(w497) -> (w496:string[][])
          }
          frame True {
            # "Get the plug-in names of all the selected files in the measurement folder"
            n200 = call "Get Selected Measurements.vi"("Tree control in"=w504, "Measurement file Tags"=w505, "error in (no error)"=w506) -> ("Tree control out"=w501:refnum<vi>, "Measurement Plug-ins"=w502:string[][], "error out"=w503:errorcluster)  [unwired: 10 in]
          }
        }
        n201 = property on="List of Selected Measurements" class="MCListbox (strict)"(error in=w482, "ItemNames"=w468, "TopLeft"=T5 {"Row"=0, "Column"=0} ("Top Left Visible Cell")) -> (error out=w480:errorcluster)  [unwired: 1 in, 1 out]
        n202 = Bundle By Name(cluster=w470, "Tree Reference"=w467, "Measurement Plug-ins"=w468) -> (w469:T3)
        n203 = Array Size(array=w468) -> (size(s)=w478:i32[])
        n204 = Index Array(array=w478) -> (element=w477:i32)  [unwired: 1 in]
        n205 = for {
          N: w477 -> [_]
          shift-right: [w491] -> w479
          shift-left: w480 -> [w492]
          i -> [w488]
          # "Set the row size for the occupied rows"
          n206 = Bundle By Name(cluster=T6 {"Row"=0, "Column"=0} ("Active Cell:Active Cell"), "Row"=w488) -> (w490:T6)
          n207 = property on="List of Selected Measurements" class="MCListbox (strict)"(error in=w492, "ActiveCell"=w490, "Height"=u32 18 ("Active Cell:Cell Size:Height")) -> (error out=w491:errorcluster)  [unwired: 1 in, 1 out]
        }
        n208 = property on="Tab Control" class="TabCtl (strict)"(error in=w479, "Value"=T1."List Plug-ins" ("Tab Control")) -> (error out=w487:errorcluster)  [unwired: 1 in, 1 out]
        n209 = call "Set Cursor Icon.vi"("Cursor icon"=u16 0, "error in (no error)"=w487) -> ("error out"=w472:errorcluster)  [unwired: 13 in]
      }
      frame "Validate plug-in rename" {
        # "Validate the name of the Plug-in after rename"
        n210 = call "Set Cursor Icon.vi"("Cursor icon"=u16 2, "error in (no error)"=w543) -> ("error out"=w535:errorcluster)  [unwired: 13 in]
        n211 = property on="List of Selected Measurements" class="MCListbox (strict)"(error in=w535) -> (error out=w527:errorcluster, "ItemNames"=w541:string[][])  [unwired: 1 in, 1 out]
        n212 = Unbundle By Name(w539) -> ("Measurement Plug-ins"=w537:string[][], "Project path"=w525:path)
        n213 = Index Array(array=w541, index (col)=1 ("disabled index (col)")) -> (element=w509:string[])  [unwired: 1 in]
        n214 = call "Get Libraries in Project.vi"("Project path"=w525, "error in (no error)"=w527) -> ("Project exists?"=w524:bool, "Library names"=w523:string[], "error out"=w526:errorcluster)  [unwired: 11 in]
        n215 = Index Array(array=w537, index (col)=1 ("disabled index (col)")) -> (element=w510:string[])  [unwired: 1 in]
        n216 = for {
          shift-right: [w549] -> w520
          shift-left: w526 -> [w550]
          tunnel: w509 -> [w547] mode=indexing
          tunnel: w524 -> [w548]
          tunnel: w523 -> [w546]
          tunnel: [w544] -> w511 mode=indexing
          tunnel: [w544] -> w507
          stop <- w545 stop-if-true
          # "Validate the plug-in names"
          n217 = call "Validate Plugin Name.vi"("Project exists?"=w548, "Library names"=w546, "Plug-in name"=w547, "error in (no error)"=w550) -> ("Valid Name?"=w544:bool, "error out"=w549:errorcluster)  [unwired: 10 in]
          n218 = Not(x=w544) -> (.not. x?=w545:bool)
        }
        n219 = Swap Values(12:w510, 13:w507, 14:w509) -> (1:w508:string[])  [unwired: 1 out]
        n220 = call "Set Plug-in Name Warning.vi"("Valid Name?"=w511, "Validated names"=w508, "error in (no error)"=w520) -> ("Warning?"=w521:bool, "error out"=w519:errorcluster)  [unwired: 11 in]
        n221 = Replace Array Subset(array=w537, new element=w508, index (col)=1 ("disabled index (col)")) -> (w512:string[][])  [unwired: 1 in]
        n222 = property on="Plug-in warning" class="Str"(error in=w519, "Visible"=w521) -> (error out=w531:errorcluster)  [unwired: 1 in, 1 out]
        n223 = Swap Values(12:u32 250 ("Size:Height"), 13:w521, 14:210 ("x")) -> (1:w522:u32)  [unwired: 1 out]
        n224 = Bundle By Name(cluster=w539, "Measurement Plug-ins"=w512) -> (w538:T3)
        n225 = property on="List of Selected Measurements" class="MCListbox (strict)"(error in=w531, "ItemNames"=w512, "Height"=w522) -> (error out=w528:errorcluster)  [unwired: 1 in, 1 out]
        n226 = Not(x=w521) -> (.not. x?=w516:bool)
        n227 = property on="Plug-in info" class="Str"(error in=w528, "Visible"=w516) -> (error out=w518:errorcluster)  [unwired: 1 in, 1 out]
        n228 = Select(t=T4."Enabled", s=w516, f=T4."Disabled and Grayed Out" ("Disabled")) -> (s? t:f=w513:T4)
        n229 = property on="Start Migration" class="Bool"(error in=w518, "DisabledEnum"=w513) -> (error out=w517:errorcluster)  [unwired: 1 in, 1 out]
        n230 = call "Set Cursor Icon.vi"("Cursor icon"=u16 0, "error in (no error)"=w517) -> ("error out"=w533:errorcluster)  [unwired: 13 in]
      }
      frame "/**********MULTIPLE MIGRATION**********/" {
      }
      frame "Update Measurement Paths" {
        w568 = 70  # Remaining Progress
        # "Update the measurement file paths for measurement folder"
        n231 = property on="Progress" class="Slide (strict)"(error in=w558, "Value"=5 ("Progress"), "Caption.Text"="Getting paths...") -> (error out=w569:errorcluster)  [unwired: 1 in, 1 out]
        n232 = Unbundle By Name(w574) -> ("Migration Status"=w562:string[][], "Measurement Plug-ins"=w564:string[][], "Measurement file/folder path"=w577:path, "Measurement Plug-ins"=w576:string[][], "Measurement folder selected?"=w575:bool)
        n233 = property on="Measurement Count" class="Slide (strict)"(error in=w569, "Value"=0 ("Measurement Count"), "Caption.Text"="Updating Measurement Paths") -> (error out=w565:errorcluster)  [unwired: 1 in, 1 out]
        n234 = Index Array(array=w564, index (col)=1 ("disabled index (col)")) -> (element=w560:string[])  [unwired: 1 in]
        n235 = call "Get Measurement Paths.vi"("Measurement Path"=w577, "Measurement Plug-ins"=w576, "Measurement folder selected?"=w575, "error in"=w565) -> ("Measurement Path Array"=w572:path[], "error out"=w554:errorcluster)  [unwired: 10 in]
        n236 = Insert Into Array(array=w562, index (col)=0 ("disabled index (col)"), new element=w560) -> (w559:string[][])  [unwired: 1 in]
        n237 = Array Size(array=w572) -> (size(s)=w567:i32)
        n238 = Quotient & Remainder(x=w568, y=w567) -> (floor(x/y)=w566:i32)  [unwired: 1 out]
        n239 = Bundle By Name(cluster=w574, "Migration Status"=w559, "Measurement File Paths"=w572, "Plugin Migration Value"=w567, "Progress per measurement"=w566) -> (w573:T3)
        n240 = property on="Progress" class="Slide (strict)"(error in=w554, "Value"=15 ("Progress")) -> (error out=w553:errorcluster)  [unwired: 1 in, 1 out]
      }
      frame "Create Project" {
        # "Check if project exists and creates a new project if not present."
        n241 = property on="Progress" class="Slide (strict)"(error in=w581, "Value"=10 ("Progress"), "Caption.Text"="Checking for project...") -> (error out=w582:errorcluster)  [unwired: 1 in, 1 out]
        n242 = property on="Measurement Count" class="Slide (strict)"(error in=w582, "Value"=10 ("Measurement Count"), "Caption.Text"="Creating project if not exist") -> (error out=w585:errorcluster)  [unwired: 1 in, 1 out]
        n243 = Unbundle By Name(w589) -> ("Project path"=w588:path)
        n244 = call "Create and Save Project.vi"("Project Path"=w588, "error in (no error)"=w585) -> ("error out"=w579:errorcluster)  [unwired: 13 in]
        n245 = property on="Progress" class="Slide (strict)"(error in=w579, "Value"=15 ("Progress")) -> (error out=w578:errorcluster)  [unwired: 1 in, 1 out]
      }
      frame "Migrate measurements" {
        # "Migrate multiple measurements along with their shared dependencies"
        n246 = property on="Progress" class="Slide (strict)"(error in=w591, "Value"=0 ("Progress")) -> (error out=w592:errorcluster)  [unwired: 1 in, 1 out]
        n247 = Unbundle By Name(w602) -> ("Project path"=w606:path, "Measurement File Paths"=w604:path[], "Measurement Plug-ins"=w607:string[][])
        n248 = property on="Measurement Count" class="Slide (strict)"(error in=w592, "Value"=20 ("Measurement Count"), "Caption.Text"="Migrating measurement(s)") -> (error out=w597:errorcluster)  [unwired: 1 in, 1 out]
        n249 = Index Array(array=w607, index (col)=1 ("disabled index (col)")) -> (element=w605:string[])  [unwired: 1 in]
        n250 = control-ref of="Progress"() -> (w590:refnum<vi>)
        n251 = call "Migrate Dependencies.vi"("Project path"=w606, "Measurement paths"=w604, "Plug-in names"=w605, "Progress"=w590, "error in"=w597) -> ("Instrument containing subVIs"=w601:path[][], "error out"=w595:errorcluster)  [unwired: 9 in]
        n252 = Bundle By Name(cluster=w602, "Instrument containing subVIs"=w601, "Measurement Progress"=30) -> (w603:T3)
        n253 = property on="Measurement Count" class="Slide (strict)"(error in=w595, "Value"=30 ("Measurement Count")) -> (error out=w594:errorcluster)  [unwired: 1 in, 1 out]
      }
      frame "Enqueue Migration Steps" {
        # "Enqueue the set of states for measurement migration"
        n254 = Unbundle By Name(w613) -> ("Plugin Migration Value"=w612:i32)
        n255 = Greater Than 0?(x=w612) -> (x > 0?=w611:bool)
        n256 = case shown="True" w611 {
          tunnel: w610 -> [w616 w623]
          tunnel: [w618 w622] -> w609
          frame False {
            # "Enqueue next step if all measurements are migrated"
            n257 = property on="Measurement Count" class="Slide (strict)"(error in=w616, "Value"=100 ("Progress")) -> (error out=w617:errorcluster)  [unwired: 1 in, 1 out]
            n258 = call "Queue Driver.vi"("States[]"=string[] ["Save Project", "Show Next Steps"], "error in (no error)"=w617, "Q Operations"=Queue_Operations."Enqueue N") -> ("error out"=w618:errorcluster)  [unwired: 11 in, 1 out]
          }
          frame True {
            # "Enqueue, if there are measurements yet to migrate"
            n259 = call "Queue Driver.vi"("States[]"=string[] ["Set Values in Dict", "Create Plugin Template", "Get Driver List", "Edit Measurement Configuration", "Edit Measurement Results", "Edit Measurement Connector Pane", "Create Wrapper", "Deserialize Cluster Data", "Add Measurement Plugin APIs", "Disable Initialize APIs", "Edit Type Specialization", "Add UI Elements", "Flatten the Clusters", "Handling Default Value", "Update Migration Count"], "error in (no error)"=w623, "Q Operations"=Queue_Operations."Enqueue N") -> ("error out"=w622:errorcluster)  [unwired: 11 in, 1 out]
          }
        }
      }
      frame "Set Values in Dict" {
        # "Measurement Status Message: Migrating 1 of N measurement(s)"
        # "Set values to the Dictionary APIs"
        n260 = Unbundle By Name(w646) -> ("Project path"=w640:path, "Instrument containing subVIs"=w636:path[][], "Measurement Plug-ins"=w645:string[][], "Migration Count"=w624:i32, "Measurement File Paths"=w633:path[])
        n261 = property on="Progress" class="Slide (strict)"(error in=w627, "Value"=0 ("Progress")) -> (error out=w632:errorcluster)  [unwired: 1 in, 1 out]
        n262 = Array Size(array=w633) -> (size(s)=w625:i32)
        n263 = Increment(x=w624) -> (x+1=w629:i32)
        n264 = Format Into String(format string="Migrating %d of %d measurement(s)", error in=w632, w629, w625) -> (resulting string=w630:string, error out=w631:errorcluster)  [unwired: 1 in]
        n265 = property on="Measurement Count" class="Slide (strict)"(error in=w631, "Caption.Text"=w630) -> (error out=w634:errorcluster)  [unwired: 1 in, 1 out]
        n266 = Index Array(array=w633, index=w624) -> (element=w643:path)
        n267 = call "Set Code Module Path.vi"("CodeModule Path"=w643, "error in (no error)"=w634) -> ("error out"=w642:errorcluster)  [unwired: 13 in]
        n268 = Index Array(array=w645, index (row)=w624, index (col)=1 ("disabled index (col)")) -> (element=w641:string)
        n269 = Index Array(array=w636, index (row)=w624) -> (element=w639:path[])  [unwired: 1 in]
        n270 = call "Set Measurement Name.vi"("Name"=w641, "error in (no error)"=w642) -> ("error out"=w638:errorcluster)  [unwired: 13 in]
        n271 = call "Set Instrument VI Paths.vi"("error in (no error)"=w638, "VI Paths[]"=w639) -> ("error out"=w637:errorcluster)  [unwired: 9 in]
        n272 = call "Set Project Path.vi"("Project Path"=w640, "error in (no error)"=w637) -> ("error out"=w626:errorcluster)  [unwired: 13 in]
      }
      frame "Create Plugin Template" {
        # "Create Measurement Plugin Template"
        n273 = property on="Progress" class="Slide (strict)"(error in=w649, "Value"=1 ("Progress"), "Caption.Text"="Creating Measurement Plugin...") -> (error out=w650:errorcluster)  [unwired: 1 in, 1 out]
        n274 = Unbundle By Name(w654) -> ("Project path"=w653:path)
        n275 = call "Create Plugin Template.vi"("Project Path"=w653, "error in (no error)"=w650) -> ("error out"=w652:errorcluster)  [unwired: 13 in]
        n276 = call "Copy Set Default Value Multiple.vi"("error in (no error)"=w652) -> ("error out"=w648:errorcluster)  [unwired: 14 in]
      }
      frame "Get Driver List" {
        # "Get the list of instrument drivers used in the measurement"
        n277 = property on="Progress" class="Slide (strict)"(error in=w656, "Value"=3 ("Progress"), "Caption.Text"="Fetching the list of instrument drivers used...") -> (error out=w657:errorcluster)  [unwired: 1 in, 1 out]
        n278 = call "List Drivers.vi"("error in (no error)"=w657) -> ("error out"=w658:errorcluster)  [unwired: 14 in]
      }
      frame "Edit Measurement Configuration" {
        # "Add elements to the measurement configuration control file"
        n279 = property on="Progress" class="Slide (strict)"(error in=w662, "Value"=4 ("Progress"), "Caption.Text"="Editing measurement configuration...") -> (error out=w663:errorcluster)  [unwired: 1 in, 1 out]
        n280 = call "Add Measurement Plugin Controls.vi"("error in (no error)"=w663) -> ("error out"=w664:errorcluster)  [unwired: 14 in]
      }
      frame "Edit Measurement Results" {
        # "Add elements to the measurement results control file"
        n281 = property on="Progress" class="Slide (strict)"(error in=w668, "Value"=5 ("Progress"), "Caption.Text"="Editing measurement results...") -> (error out=w669:errorcluster)  [unwired: 1 in, 1 out]
        n282 = call "Add Meas Plugin Indicators.vi"("error in (no error)"=w669) -> ("error out"=w670:errorcluster)  [unwired: 14 in]
      }
      frame "Edit Measurement Connector Pane" {
        # "Edit the connector pane of the duplicated measurement"
        n283 = property on="Progress" class="Slide (strict)"(error in=w674, "Value"=6 ("Progress"), "Caption.Text"="Editing the connector pane of the measurement...") -> (error out=w675:errorcluster)  [unwired: 1 in, 1 out]
        n284 = call "Edit Connector Pane Multiple.vi"("error in (no error)"=w675) -> ("error out"=w676:errorcluster)  [unwired: 14 in]
      }
      frame "Create Wrapper" {
        # "Create a wrapper for the measurement"
        n285 = property on="Progress" class="Slide (strict)"(error in=w680, "Value"=7 ("Progress"), "Caption.Text"="Creating wrapper for the measurement...") -> (error out=w681:errorcluster)  [unwired: 1 in, 1 out]
        n286 = call "Create Wrapper for Measurement Plugin.vi"("error in (no error)"=w681) -> ("error out"=w682:errorcluster)  [unwired: 14 in]
      }
      frame "Deserialize Cluster Data" {
        # "Deserialize the connection in the wrapper vi"
        n287 = property on="Progress" class="Slide (strict)"(error in=w686, "Value"=8 ("Progress"), "Caption.Text"="Flattening and unflattening the cluster data in Wrapper...") -> (error out=w687:errorcluster)  [unwired: 1 in, 1 out]
        n288 = call "Deserialize Connections in Wrapper Plugin.vi"("error in (no error)"=w687) -> ("error out"=w688:errorcluster)  [unwired: 14 in]
      }
      frame "Add Measurement Plugin APIs" {
        # "Add all the rquired Measurement Plugin APIs in measurement logic and wire them appropriately"
        n289 = property on="Progress" class="Slide (strict)"(error in=w692, "Value"=9 ("Progress"), "Caption.Text"="Editing measurement logic...") -> (error out=w693:errorcluster)  [unwired: 1 in, 1 out]
        n290 = call "Create Measurement Plugin subVIs.vi"("error in (no error)"=w693) -> ("error out"=w694:errorcluster)  [unwired: 14 in]
      }
      frame "Disable Initialize APIs" {
        # "Disable the initialize and close in the measurement"
        n291 = property on="Progress" class="Slide (strict)"(error in=w698, "Value"=10 ("Progress"), "Caption.Text"="Disabling and removing the Initalize and Close APIs...") -> (error out=w699:errorcluster)  [unwired: 1 in, 1 out]
        n292 = call "Add Diagram disable structure.vi"("error in (no error)"=w699) -> ("error out"=w700:errorcluster)  [unwired: 14 in]
      }
      frame "Edit Type Specialization" {
        # "Edit the Type Specializations.vi"
        n293 = property on="Progress" class="Slide (strict)"(error in=w704, "Value"=11 ("Progress"), "Caption.Text"="Editing the Type Specialization VI...") -> (error out=w705:errorcluster)  [unwired: 1 in, 1 out]
        n294 = call "Edit Plugin Type Specialization.vi"("error in (no error)"=w705) -> ("error out"=w706:errorcluster)  [unwired: 14 in]
      }
      frame "Add UI Elements" {
        # "Edit the Measurement UI.vi"
        n295 = property on="Progress" class="Slide (strict)"(error in=w710, "Value"=12 ("Progress"), "Caption.Text"="Editing Measurement UI...") -> (error out=w711:errorcluster)  [unwired: 1 in, 1 out]
        n296 = call "Add Elements to Meas Plugin UI.vi"("error in (no error)"=w711) -> ("error out"=w712:errorcluster)  [unwired: 14 in]
      }
      frame "Flatten the Clusters" {
        # "Creating string ande serialize data for the wrapper connections"
        n297 = property on="Progress" class="Slide (strict)"(error in=w716, "Value"=13 ("Progress"), "Caption.Text"="Creating events and flatten the data...") -> (error out=w717:errorcluster)  [unwired: 1 in, 1 out]
        n298 = call "Create String and Serialize Cluster Data in UI.vi"("error in (no error)"=w717) -> ("error out"=w718:errorcluster)  [unwired: 14 in]
      }
      frame "Handling Default Value" {
        # "Setting default value for cluster based on string controls"
        n299 = property on="Progress" class="Slide (strict)"(error in=w722, "Value"=14 ("Progress"), "Caption.Text"="Loading values for string controls in UI...") -> (error out=w723:errorcluster)  [unwired: 1 in, 1 out]
        n300 = call "Logic for Default Case Multiple.vi"("error in (no error)"=w723) -> ("error out"=w724:errorcluster)  [unwired: 14 in]
      }
      frame "Save Project" {
        # "Saving the project and libraries"
        n301 = property on="Progress" class="Slide (strict)"(error in=w728, "Value"=15 ("Progress"), "Caption.Text"="Saving the project files...") -> (error out=w730:errorcluster)  [unwired: 1 in, 1 out]
        n302 = call "Save Projects and Libraries.vi"("error in (no error)"=w730) -> ("error out"=w729:errorcluster)  [unwired: 10 in]
      }
      frame "Update Migration Count" {
        # "Updating the migration count and migration status"
        n303 = in-place {
          in-place-border: [w741] -> w735
          n304 = in-place-cluster #2(w740) -> ("Plugin Migration Value"=w753:i32, "Migration Count"=w744:i32, "Measurement Progress"=w751:i32, "Progress per measurement"=w750:i32, "Migration Status"=w747:string[][])
          n305 = Index Array(array=w747, index (col)=1 ("disabled index (col)")) -> (element=w745:string[])  [unwired: 1 in]
          n306 = Insert Into Array(array=w745, index=w744, new element="Success") -> (w742:string[])
          n307 = Insert Into Array(array=w747, index (col)=1 ("disabled index (col)"), new element=w742) -> (w749:string[][])  [unwired: 1 in]
          n308 = Increment(x=w744) -> (x+1=w754:i32)
          n309 = Add(x=w751, y=w750) -> (x+y=w741:i32)
          n310 = Decrement(x=w753) -> (x-1=w752:i32)
          n311 = in-place-cluster #2("Plugin Migration Value"=w752, "Migration Count"=w754, "Measurement Progress"=w741, "Progress per measurement"=w750, "Migration Status"=w749) -> (w739:T3)
        }
        n312 = property on="Measurement Count" class="Slide (strict)"(error in=w734, "Value"=w735) -> (error out=w733:errorcluster)  [unwired: 1 in, 1 out]
        n313 = call "Queue Driver.vi"("State"="Enqueue Migration Steps", "error in (no error)"=w733, "Q Operations"=Queue_Operations."Enqueue") -> ("error out"=w738:errorcluster)  [unwired: 11 in, 1 out]
      }
      frame "Update count on Fail" {
        # "Updating the migration count and migration status"
        n314 = in-place {
          in-place-border: [w763] -> w757
          n315 = in-place-cluster #3(w762) -> ("Plugin Migration Value"=w775:i32, "Migration Count"=w766:i32, "Measurement Progress"=w773:i32, "Progress per measurement"=w772:i32, "Migration Status"=w769:string[][])
          n316 = Index Array(array=w769, index (col)=1 ("disabled index (col)")) -> (element=w767:string[])  [unwired: 1 in]
          n317 = Insert Into Array(array=w767, index=w766, new element="Fail") -> (w764:string[])
          n318 = Insert Into Array(array=w769, index (col)=1 ("disabled index (col)"), new element=w764) -> (w771:string[][])  [unwired: 1 in]
          n319 = Increment(x=w766) -> (x+1=w776:i32)
          n320 = Add(x=w773, y=w772) -> (x+y=w763:i32)
          n321 = Decrement(x=w775) -> (x-1=w774:i32)
          n322 = in-place-cluster #3("Plugin Migration Value"=w774, "Migration Count"=w776, "Measurement Progress"=w763, "Progress per measurement"=w772, "Migration Status"=w771) -> (w761:T3)
        }
        n323 = property on="Measurement Count" class="Slide (strict)"(error in=w756, "Value"=w757) -> (error out=w755:errorcluster)  [unwired: 1 in, 1 out]
        n324 = call "Queue Driver.vi"("State"="Enqueue Migration Steps", "error in (no error)"=w755, "Q Operations"=Queue_Operations."Enqueue") -> ("error out"=w760:errorcluster)  [unwired: 11 in, 1 out]
      }
      frame "/**********NEXT STEPS POST MIGRATION**********/" {
      }
      frame "Show Next Steps" {
        # "To change unwanted loading symbol"
        # "Showing the migration status"
        n325 = in-place {
          in-place-border: [w802] -> w786
          n326 = in-place-cluster #4(w794) -> ("Migration Status"=w803:string[][])
          n327 = Index Array(array=w803, index (col) #1=0 ("disabled index (col)"), index (col) #2=1 ("index (col)")) -> (element #1=w806:string[], element #2=w804:string[])  [unwired: 2 in]
          n328 = for {
            tunnel: w806 -> [_] mode=indexing
            tunnel: w804 -> [w813]
            shift-right: [w808] -> w802
            shift-left: w803 -> [w811]
            i -> [w810]
            n329 = Index Array(array=w813, index=w810) -> (element=w812:string)
            n330 = Empty String/Path?(string/path=w812) -> (empty?=w809:bool)
            n331 = case shown="True" w809 {
              tunnel: w811 -> [w814 w821]
              tunnel: w810 -> [_ w818]
              tunnel: [w814 w822] -> w808
              frame False {
              }
              frame True {
                # "Insert 'Fail' for empty status"
                n332 = Index Array(array=w821, index (col)=1 ("disabled index (col)")) -> (element=w819:string[])  [unwired: 1 in]
                n333 = Insert Into Array(array=w819, index=w818, new element="Fail" ("new element/subarray")) -> (w816:string[])
                n334 = Insert Into Array(array=w821, index (col)=1 ("disabled index (col)"), new element=w816) -> (w822:string[][])  [unwired: 1 in]
              }
            }
          }
          n335 = in-place-cluster #4("Migration Status"=w802) -> (w793:T3)
        }
        n336 = property on="Tab Control" class="TabCtl (strict)"(error in=w789, "Value"=T1."Status" ("Tab Control")) -> (error out=w791:errorcluster)  [unwired: 1 in, 1 out]
        n337 = property on="Migration Status" class="MCListbox (strict)"(error in=w791, "Allow Editing Cells"=FALSE) -> (error out=w790:errorcluster)  [unwired: 1 in, 1 out]
        n338 = property on="Migration Status" class="MCListbox (strict)"(error in=w790, "ItemNames"=w786) -> (error out=w781:errorcluster)  [unwired: 1 in, 1 out]
        n339 = Index Array(array=w786, index (col)=1 ("disabled index (col)")) -> (element=w784:string[])  [unwired: 1 in]
        n340 = Equal?(x=w784, y="Fail" ("new element/subarray")) -> (x = y?=w782:bool[])
        n341 = And Array Elements(Boolean array=w782) -> (logical AND=w779:bool)
        n342 = case "All the measurements failed?" shown="True" w779 {
          tunnel: w781 -> [w797 w801]
          tunnel: [w798 w800] -> w780
          frame False {
            n343 = property on="Review" class="Bool"(error in=w797, "BoolText.Text"="Review Plug-ins" ("Boolean Text.Text")) -> (error out=w798:errorcluster)  [unwired: 1 in, 1 out]
          }
          frame True {
            # "Change Bool Text to Start next migration"
            n344 = property on="Review" class="Bool"(error in=w801, "BoolText.Text"="Start Next Migration" ("Boolean Text.Text")) -> (error out=w800:errorcluster)  [unwired: 1 in, 1 out]
          }
        }
        n345 = call "Set Cursor Icon.vi"("Cursor icon"=u16 0, "error in (no error)"=w780) -> ("error out"=w788:errorcluster)  [unwired: 13 in]
      }
      frame "Show Links" {
        # "Showing links for the migrated measurements"
        n346 = Unbundle By Name(w830) -> ("Migration Status"=w832:string[][])
        n347 = for {
          tunnel: w832 -> [w839] mode=indexing
          tunnel: [w833] -> w827 mode=indexing if=w836
          # "Populating combo box with successfully migrated plugin names"
          n348 = Index Array(array=w839, index #1=0 ("index"), index #2=1 ("index")) -> (element #1=w833:string, element #2=w834:string)
          n349 = Equal?(x=w834, y="Success") -> (x = y?=w836:bool)
        }
        n350 = Index Array(array=w827, index=0) -> (element=w823:string)
        n351 = property on="Select Plug-in" class="CmbBox"(error in=w831, "Strings[]"=w827, "Value"=w823) -> (error out=w825:errorcluster)  [unwired: 1 in, 1 out]
        n352 = call "Set Measurement Name.vi"("Name"=w823, "error in (no error)"=w825) -> ("error out"=w824:errorcluster)  [unwired: 13 in]
        n353 = property on="Tab Control" class="TabCtl (strict)"(error in=w824, "Value"=T1."Links" ("Tab Control")) -> (error out=w828:errorcluster)  [unwired: 1 in, 1 out]
      }
      frame "/**********ERROR**********/" {
      }
      frame "Error" {
        # "Handle the error and alert user"
        n354 = call <vilib>:"Clear Errors.vi"("error in (no error)"=w849) -> ("error out"=w850:errorcluster)  [unwired: 5 in, 1 out]
        n355 = Equal?(x=string[] ["Set Values in Dict", "Create Plugin Template", "Get Driver List", "Edit Measurement Configuration", "Edit Measurement Results", "Edit Measurement Connector Pane", "Create Wrapper", "Deserialize Cluster Data", "Add Measurement Plugin APIs", "Disable Initialize APIs", "Edit Type Specialization", "Add UI Elements", "Flatten the Clusters", "Handling Default Value", "Update Migration Count"] ("States[]"), y=w842) -> (x = y?=w844:bool[])
        n356 = call "Queue Driver.vi"("error in (no error)"=w850, "Q Operations"=Queue_Operations."Flush") -> ("error out"=w847:errorcluster)  [unwired: 12 in, 1 out]
        n357 = Or Array Elements(Boolean array=w844) -> (logical OR=w843:bool)
        n358 = case shown="True" w843 {
          tunnel: w847 -> [w857 w869]
          tunnel: [w856 w867] -> w846
          tunnel: w842 -> [w855 _]
          frame False {
            # "If error occurs in other steps"
            n359 = Equal?(x=string[] ["Update Measurement Paths", "Create Project", "Migrate measurements"] ("States[]"), y=w855) -> (x = y?=w853:bool[])
            n360 = Or Array Elements(Boolean array=w853) -> (logical OR=w852:bool)
            n361 = case "Error in Migration?" shown="False" w852 {
              tunnel: w857 -> [w861 w864]
              tunnel: [w860 w863] -> w856
              frame False {
                # "Restart Migration tool"
                n362 = call "Queue Driver.vi"("States[]"=string[] ["Reinitialize", "Initialize UI", "Populate project path"], "error in (no error)"=w861, "Q Operations"=Queue_Operations."Enqueue N") -> ("error out"=w860:errorcluster)  [unwired: 11 in, 1 out]
              }
              frame True {
                # "Show Next steps"
                n363 = call "Queue Driver.vi"("State"="Show Next Steps", "error in (no error)"=w864, "Q Operations"=Queue_Operations."Enqueue") -> ("error out"=w863:errorcluster)  [unwired: 11 in, 1 out]
              }
            }
          }
          frame True {
            # "If error occurs during measurement migration"
            n364 = call "Queue Driver.vi"("State"="Update count on Fail", "error in (no error)"=w869, "Q Operations"=Queue_Operations."Enqueue") -> ("error out"=w867:errorcluster)  [unwired: 11 in, 1 out]
          }
        }
      }
      frame "/**********EXIT**********/" {
      }
      frame "Exit" {
        # "Flush the queue elements and stop execution"
        n365 = call "Queue Driver.vi"("error in (no error)"=w882, "Q Operations"=Queue_Operations."Flush") -> ("error out"=w876:errorcluster)  [unwired: 12 in, 1 out]
        n366 = call "Queue Driver.vi"("error in (no error)"=w876, "Q Operations"=Queue_Operations."Release") -> ("error out"=w875:errorcluster)  [unwired: 12 in, 1 out]
        n367 = Unbundle By Name(w880) -> ("Tree Reference"=w879:refnum<vi>)
        n368 = Close Reference(reference=w879, error in (no error)=w875) -> (error out=w873:errorcluster)
        n369 = call "Dictionary.vi"("error in (no error)"=w873, "Dict States"=Dictionary_States."Delete All") -> ("error out"=w872:errorcluster)  [unwired: 12 in, 1 out]
      }
    }
  }
  n370 = disable-structure shown="Disabled" {
    disable-tunnel: w3 -> [w884 _]
    disable-tunnel: [w883 _] -> w2
    frame Disabled {
      n371 = invoke class="VI" method="FP.Close"(error in=w884) -> (error out=w883:errorcluster)  [unwired: 2 in, 2 out]
    }
    frame Enabled {
    }
  }
  "error out" <- w2
